vi "Emulate aquisition.vi"() -> ()   [LabVIEW 2020]
uses:
  controls/Acquisition data --typedef.ctl
  controls/Graph data --typedef.ctl
  controls/Color --typedef.ctl
panel:
  out "J-EFf I":cluster{dbl[], dbl[]}(graph) caption="L-V"
  out "I-V":cluster{dbl[], dbl[]}(graph) caption="L-V"
  out "L-V 2":cluster{dbl[], dbl[]}(graph) caption="L-V"
  in  "Color":T1
  in  "OLED A":dbl=0.07 caption="Area del OLED [cm2]"
  in  "OLED-PD dist":dbl=1.0 caption="Distancia OLED-fotodiodo [cm]"
  out "EFf I-V":cluster{dbl[], dbl[]}(graph) caption="L-V"
  out "Eff L-V":cluster{dbl[], dbl[]}(graph) caption="L-V"
  out "L-V":cluster{dbl[], dbl[]}(graph)
  out "J-V":cluster{dbl[], dbl[]}(graph)
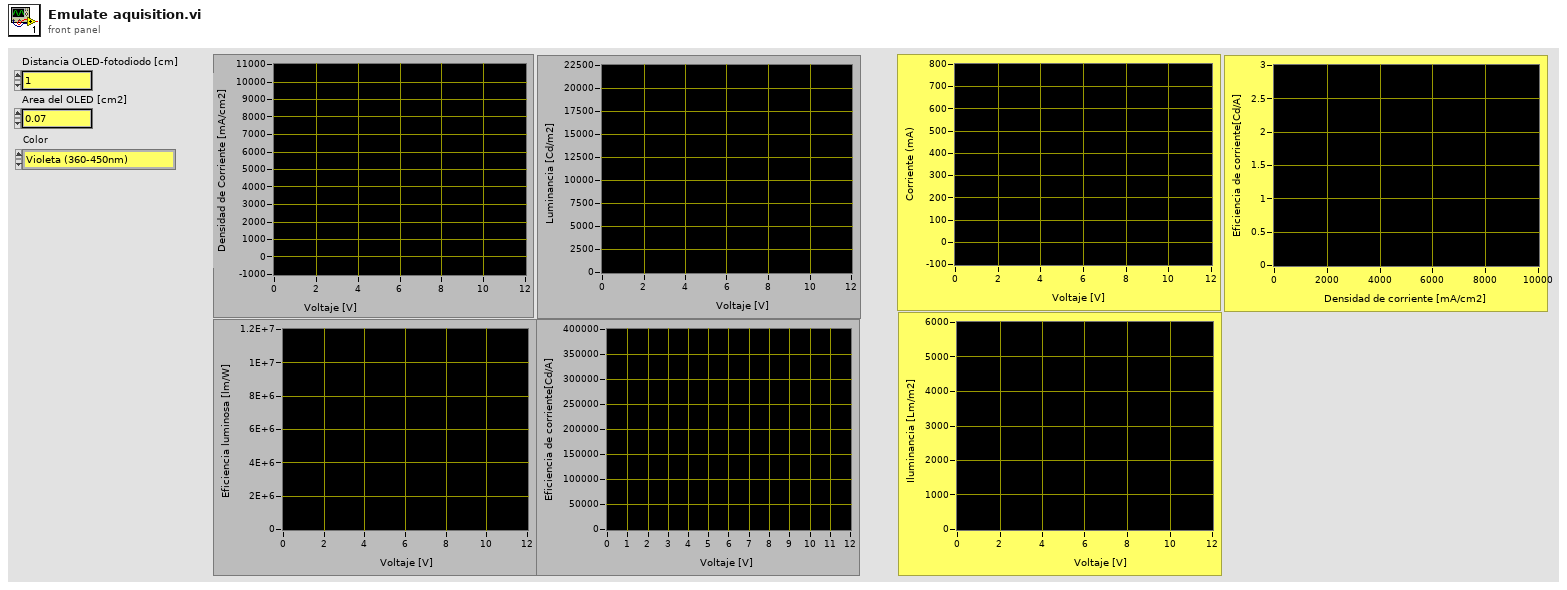
[diagram p1: front panel]
types:
  T1 = typedef "Color --typedef.ctl" = enum16{"Violeta (360-450nm)", "Azul (450-500nm)", "Verde(500-570nm)", "Amarillo (570-590nm)", "Naranja (600-610nm)", "Rojo (610-670nm)", "Blanco"}
  T2 = typedef "Graph data --typedef.ctl" = cluster{"Voltaje [V]":dbl[], "Corriente [mA]":dbl[], "Densidad de corriente [CD/A]":dbl[], "Iluminancia [Lm/m2]":dbl[], "Luminance [Cd/m2]":dbl[], "Ef corriente [Cd/A]":dbl[], "Ef Luminosa [Cd/W]":dbl[], "V detector [V]":dbl[], "Pin [W]":dbl[]}
  T3 = typedef "Acquisition data --typedef.ctl" = cluster{"Iluminancia  lm/m2":dbl, "DAQ AV":dbl, "Luminancia (Cd/m2)":dbl, "Pin(W)":dbl, "SM V":dbl, "SM I":dbl, "OLED Area cm2":dbl}
  T4 = cluster{"Voltaje [V]":dbl[], "Iluminancia [Lm/m2]":dbl[]}
  T5 = cluster{"Voltaje [V]":dbl[], "Densidad de corriente [CD/A]":dbl[]}
  T6 = cluster{"Voltaje [V]":dbl[], "Luminance [Cd/m2]":dbl[]}
  T7 = cluster{"Voltaje [V]":dbl[], "Ef corriente [Cd/A]":dbl[]}
  T8 = cluster{"Voltaje [V]":dbl[], "Ef Luminosa [Cd/W]":dbl[]}
  T9 = cluster{"Voltaje [V]":dbl[], "Corriente [mA]":dbl[]}
  T10 = cluster{"Densidad de corriente [CD/A]":dbl[], "Ef corriente [Cd/A]":dbl[]}
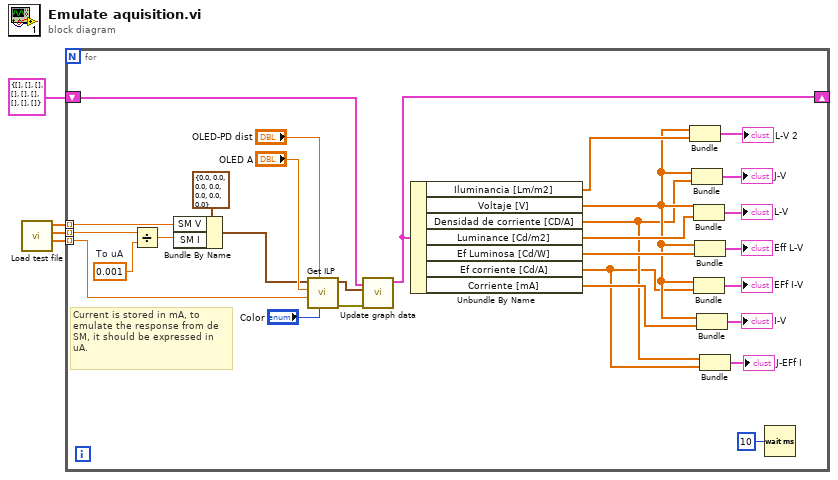
[diagram p0: block diagram]
diagram:
  n1 = call "Load test file.vi"() -> ("Voltaje del detector [V]"=w2:dbl[], "Corriente [mA]"=w3:dbl[], "Voltaje [V]"=w4:dbl[])  [unwired: 9 in]
  n2 = for {
    tunnel: w4 -> [w24] mode=indexing
    tunnel: w3 -> [w23] mode=indexing
    tunnel: w2 -> [w21] mode=indexing
    shift-right: [w17] -> _
    shift-left: T2 {"Voltaje [V]"=[], "Corriente [mA]"=[], "Densidad de corriente [CD/A]"=[], "Iluminancia [Lm/m2]"=[], "Luminance [Cd/m2]"=[], "Ef corriente [Cd/A]"=[], "Ef Luminosa [Cd/W]"=[], "V detector [V]"=[], "Pin [W]"=[]} ("Graph data") -> [w18]
    w14 = 0.001  # To uA
    # "Current is stored in mA, to emulate the response from de SM, it should be expressed in uA."
    n3 = Divide(x=w23, y=w14) -> (x/y=w15:dbl)
    n4 = Bundle By Name(cluster=T3 {"Iluminancia  lm/m2"=0.0, "DAQ AV"=0.0, "Luminancia (Cd/m2)"=0.0, "Pin(W)"=0.0, "SM V"=0.0, "SM I"=0.0, "OLED Area cm2"=0.0} ("Acquistion Data"), "SM V"=w24, "SM I"=w15) -> (w22:T3)
    n5 = call "Get ILP.vi"("Color"="Color", "OLED-PD dist"="OLED-PD dist", "DAQ V"=w21, "OLED A"="OLED A", "Acquistion Data"=w22) -> ("error out"=w20:errorcluster, "Acquistion Data"=w19:T3)  [unwired: 5 in]
    n6 = call "Update graph data.vi"("error in (no error)"=w20, "Acquisition data"=w19, "Graph data"=w18) -> ("Graph data"=w17:T2)  [unwired: 7 in, 1 out]
    n7 = Unbundle By Name(w17) -> ("Iluminancia [Lm/m2]"=w11:dbl[], "Voltaje [V]"=w9:dbl[], "Densidad de corriente [CD/A]"=w6:dbl[], "Luminance [Cd/m2]"=w29:dbl[], "Ef Luminosa [Cd/W]"=w28:dbl[], "Ef corriente [Cd/A]"=w5:dbl[], "Corriente [mA]"=w8:dbl[])
    n8 = Bundle("Voltaje [V]"=w9, "Iluminancia [Lm/m2]"=w11) -> (→"L-V 2":T4)  [unwired: 1 in]
    n9 = Bundle("Voltaje [V]"=w9, "Densidad de corriente [CD/A]"=w6) -> (→"J-V":T5)  [unwired: 1 in]
    n10 = Bundle("Voltaje [V]"=w9, "Luminance [Cd/m2]"=w29) -> (→"L-V":T6)  [unwired: 1 in]
    n11 = Bundle("Voltaje [V]"=w9, "Ef corriente [Cd/A]"=w5) -> (→"EFf I-V":T7)  [unwired: 1 in]
    n12 = Bundle("Voltaje [V]"=w9, "Ef Luminosa [Cd/W]"=w28) -> (→"Eff L-V":T8)  [unwired: 1 in]
    n13 = Bundle("Voltaje [V]"=w9, "Corriente [mA]"=w8) -> (→"I-V":T9)  [unwired: 1 in]
    n14 = Bundle("Densidad de corriente [CD/A]"=w6, "Ef corriente [Cd/A]"=w5) -> (→"J-EFf I":T10)  [unwired: 1 in]
    n15 = Wait (ms)(milliseconds to wait=u32 10) -> ()  [unwired: 1 out]
  }
